vi "Cleanup Session.vi"(8 "error in":errorcluster, 11 "Plugin in":refnum<class "Nominal-TDMS-Upload.lvclass">) -> (0 "error out":errorcluster, 3 "Plugin out":refnum<class "Nominal-TDMS-Upload.lvclass">)   [LabVIEW 2026, in "Nominal-TDMS-Upload.lvlib" / "Nominal-TDMS-Upload.lvclass"]
uses:
  Nominal-TDMS-Upload.lvclass
  Nominal-TDMS-Upload.lvclass/Nominal-TDMS-Upload.ctl
  <vilib>/Nominal/Nominal IO Client/lv_src/Nominal Client/Nominal Client.lvclass/Nominal Client.ctl
  <vilib>/Nominal/Nominal IO Client/lv_src/Nominal Client/Nominal Client.lvclass
  <vilib>/Nominal/Nominal IO Client/submodules/nominal-streaming-labview-ffi/lv_src/Stream/Stream.lvclass
  <vilib>/Nominal/Nominal IO Client/submodules/nominal-streaming-labview-ffi/lv_src/Channel/Channel.lvclass
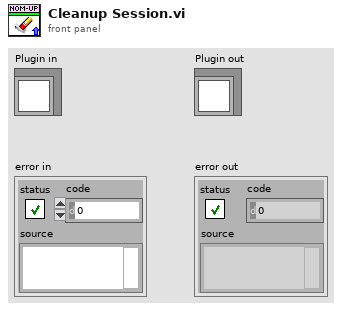
[diagram p1: front panel]
types:
  T1 = typedef "Nominal-TDMS-Upload.lvlib/Nominal-TDMS-Upload.lvclass/stream reference data.ctl" = cluster{"Nominal Client":refnum<class "Nominal Client.lvclass">, "Dataset":refnum<class "dataset.lvclass">, "dataset stream":refnum<class "Stream.lvclass">, "Map":map{string, refnum<class "Channel.lvclass">}}
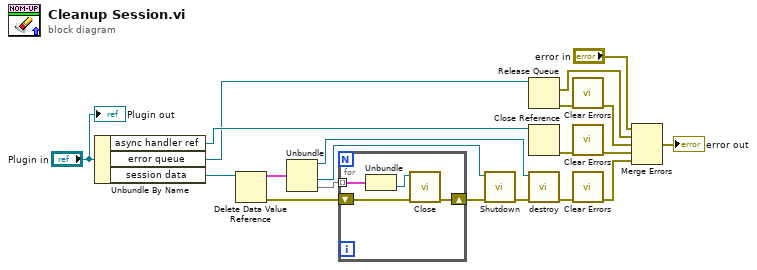
[diagram p0: block diagram]
diagram:
  n1 = Unbundle By Name("Plugin in") -> ("async handler ref"=w17:refnum<vi>, "error queue"=w15:refnum<queue>, "session data"=w10:refnum<data-value>)
  n2 = Delete Data Value Reference(data value reference=w10) -> (data value=w9:T1, error out=w5:errorcluster)  [unwired: 1 in]
  n3 = Unbundle(w9) -> ("Nominal Client"=w7:refnum<class "Nominal Client.lvclass">, "dataset stream"=w6:refnum<class "Stream.lvclass">, "Map"=w8:map{string, refnum<class "Channel.lvclass">})  [unwired: 1 out]
  n4 = for {
    shift-right: [w24] -> w11
    shift-left: w5 -> [w23]
    tunnel: w8 -> [w22] mode=indexing
    n5 = Unbundle(w22) -> ("channel"=w21:refnum<class "Channel.lvclass">)  [unwired: 1 out]
    n6 = call <vilib>:"Close.vi"("error in (no error)"=w23, "Channel in"=w21) -> ("error out"=w24:errorcluster)  [unwired: 9 in]
  }
  n7 = call <vilib>:"Shutdown.vi"("error in (no error)"=w11, "Nominal Streaming in"=w6) -> ("error out"=w12:errorcluster)  [unwired: 8 in, 1 out]
  n8 = Release Queue(queue=w15) -> (remaining elements=w14:errorcluster[], error out=w13:errorcluster)  [unwired: 2 in, 1 out]
  n9 = Close Reference(reference=w17) -> (error out=w16:errorcluster)  [unwired: 1 in]
  n10 = call <vilib>:"destroy.vi"("error in"=w12, "Nominal Client"=w7) -> ("error out"=w4:errorcluster)  [unwired: 9 in]
  n11 = call <vilib>:"Clear Errors.vi"("error in (no error)"=w13) -> ("error out"=w1:errorcluster)  [unwired: 5 in, 1 out]
  n12 = call <vilib>:"Clear Errors.vi"("error in (no error)"=w16) -> ("error out"=w2:errorcluster)  [unwired: 5 in, 1 out]
  n13 = call <vilib>:"Clear Errors.vi"("error in (no error)"=w4) -> ("error out"=w3:errorcluster)  [unwired: 5 in, 1 out]
  n14 = Merge Errors("error in", w14, w1, w2, w3) -> (→"error out":errorcluster)
  "Plugin out" <- "Plugin in"
